vi "Modbus Strings.vi"() -> ()   [LabVIEW 2026, in "Modbus.lvlib" / "Modbus.lvclass"]
uses:
  Modbus.lvclass
panel:
  in  "Not connected":string="Not connected"
  in  "Connected":string="Connected"
  in  "Str In Name":string="String Input %d"
  in  "Str In ID":string="Str In%d"
  in  "Bool Out Name":string="Boolean Ouput %d"
  in  "Bool In Name":string="Boolean Input %d"
  in  "Bool Out ID":string="Bool Out%d"
  in  "Bool In ID":string="Bool In%d"
  in  "Num Out Name":string="Numeric Output %d"
  in  "Num In Name":string="Numeric Input %d"
  in  "Num Out ID":string="Num Out%d"
  in  "Num In ID":string="Num In%d"
  in  "Connection Name":string="Connection Settings"
  in  "Connection ID":string="Connection"
  in  "Timeout":string="Connection timeout (ms)"
  in  "Address":string="Address"
  in  "Byte Location":string="Byte location"
  in  "Size":string="Size"
  in  "Boolean Outputs":string="Write Boolean channels"
  in  "String Inputs":string="Read string channels"
  in  "Boolean Inputs":string="Read Boolean channels"
  in  "Numeric Outputs":string="Write numeric channels"
  in  "Numeric Inputs":string="Read numeric channels"
  in  "Signed Rep":string="Signed integer representation"
  in  "Order":string="Multi-register order"
  in  "Port":string="Port"
  in  "Outputs":string="Write"
  in  "Data Type":string="Data type"
  in  "Number of Registers to Read":string="Number of registers to read"
  in  "Starting Address":string="Starting address"
  in  "Modbus Table":string="Modbus table"
  in  "Inputs":string="Read"
  in  "Period":string="Polling period (ms)"
  in  "IP Address":string="Modbus server IP address"
  # "Device Properties:"
  # "Connection Properties:"
  # "I/O Channel Names/Sections::"
  # "I/O Channel Properties::"
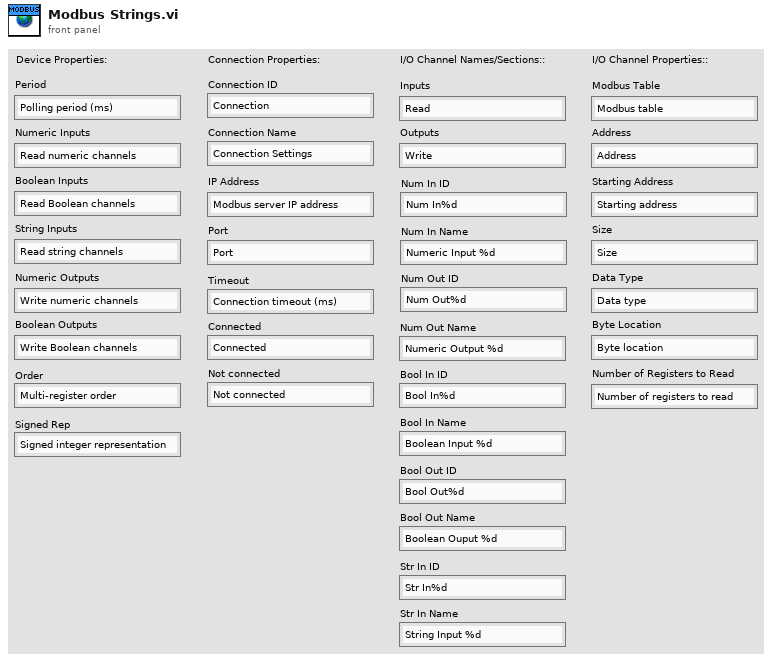
[diagram p1: front panel]
diagram:
